vi "GetDevAddress.vi"(1 "DevNum":u32=10, 2 "DevType":enum16{"LAN", "USB"}(ring)=enum."USB", 3 "UCI_DllPath":path) -> (0 "DevAddressGroup":string[](array[string]))   [LabVIEW 2015]
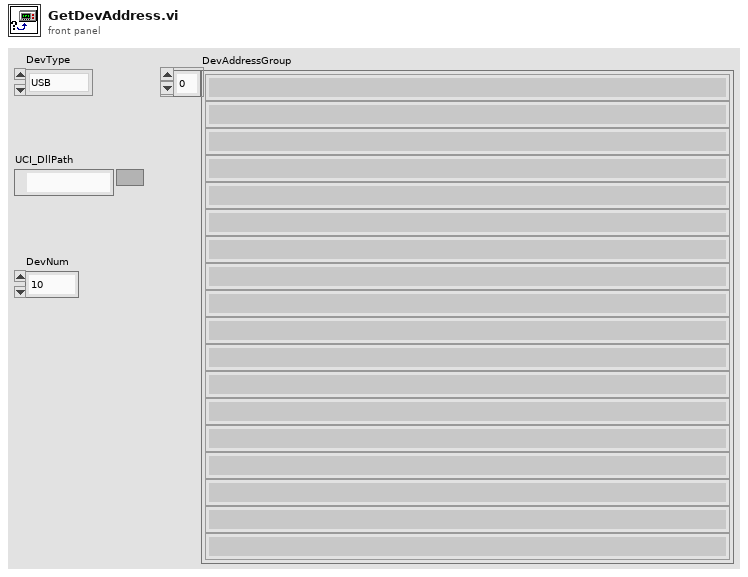
[diagram p1: front panel]
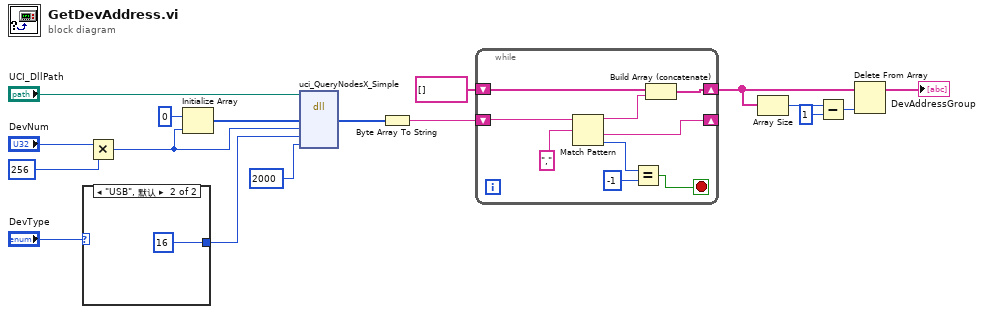
[diagram p0: block diagram]
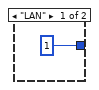
[diagram p2: hidden frame]
diagram:
  n1 = case shown="\"USB\", 默认" "DevType" {
    tunnel: [u32 1 u32 16] -> w6
    frame "LAN" {
    }
    frame "USB", Default {
    }
  }
  n2 = Multiply(x="DevNum", y=u32 256) -> (x*y=w4:u32)
  n3 = Initialize Array(u8 0 ("元素"), w4) -> (w15:u8[])
  n4 = dll-call lib="E:/JL-Project/LabView-Project/ASCII/uci.dll" fn="uci_QueryNodesX_Simple"(path in="UCI_DllPath", "_addr_msg"=w15, "_addr_msg_len"=w4, "_node_type"=w6, "_timeout"=u32 2000) -> ("_addr_msg"=w14:u8[])  [unwired: 6 in, 2 out]
  n5 = Byte Array To String(unsigned byte array=w14) -> (string=w7:string)
  n6 = while {
    shift-right: [w24] -> _
    shift-left: w7 -> [w25]
    shift-right: [w21] -> w12
    shift-left: string[] [] -> [w22]
    stop <- w26 stop-if-true
    n7 = Match Pattern(string=w25, regular expression="," ("正则表达式")) -> (before substring=w23:string, after substring=w24:string, offset past match=w28:i32)  [unwired: 1 in, 1 out]
    n8 = Equal?(x=w28, y=-1) -> (x = y?=w26:bool)
    n9 = Build Array (concatenate)(w22, w23) -> (w21:string[])
  }
  n10 = Array Size(array=w12) -> (size(s)=w10:i32)
  n11 = Subtract(x=w10, y=1) -> (x-y=w8:i32)
  n12 = Delete From Array(array=w12, index=w8) -> (array with subset deleted=→"DevAddressGroup":string[])  [unwired: 1 in, 1 out]
